vi "Base Probability calculation.vi"(8 "std [%]":dbl=0.02 format="%#_13g", 10 "Base Ex Info":T1, 11 "Relative Array":dbl[](array[numeric])) -> (3 "Time Probability":dbl[][](array[numeric]))   [LabVIEW 2018]
uses:
  <vilib>/gmath/statdist.llb/Normal PDF.vi
  <vilib>/gmath/NI_Gmath.lvlib
panel:
  out "Base R level":dbl[](array[numeric])
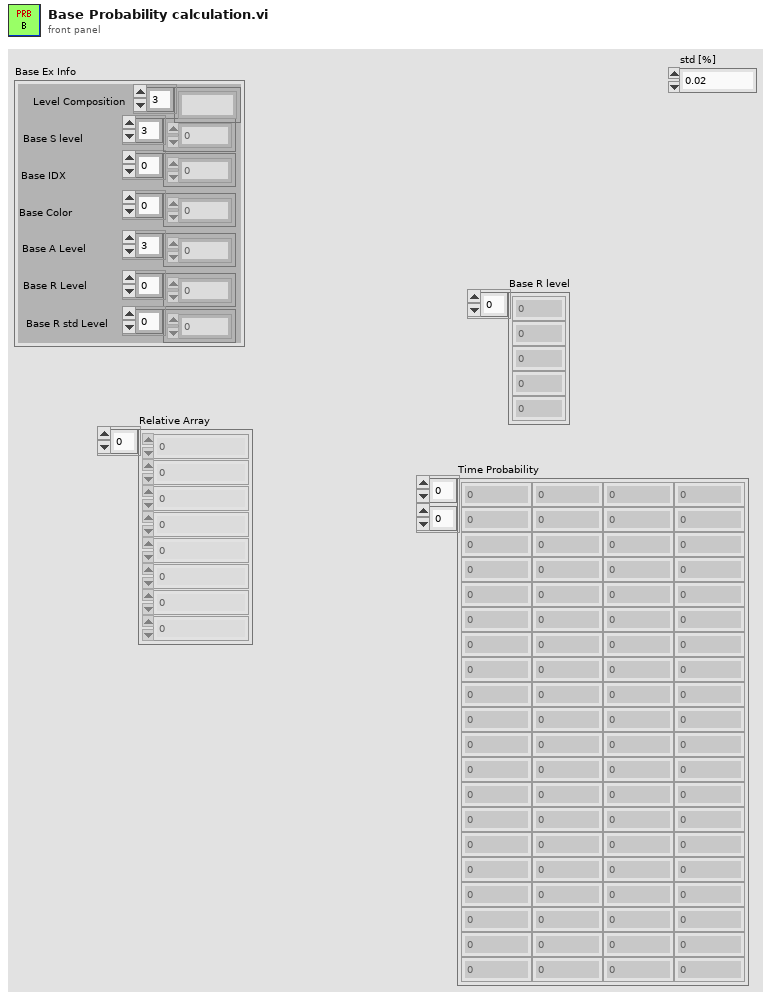
[diagram p1: front panel]
types:
  T1 = cluster{"Level Composition":string[], "Base S level":dbl[], "Base IDX":i32[], "Base Color":u32[], "Base A Level":dbl[], "Base R Level":dbl[], "Base R std Level":dbl[]}
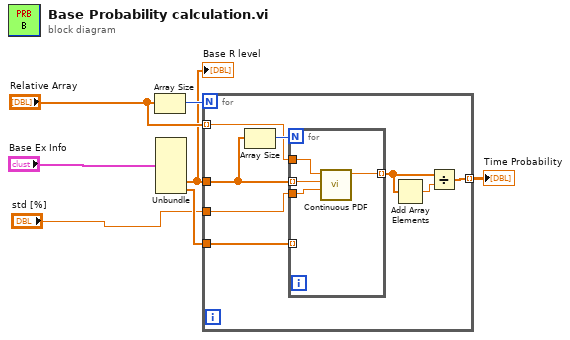
[diagram p0: block diagram]
diagram:
  n1 = Array Size(array="Relative Array") -> (size(s)=w7:i32)
  n2 = Unbundle("Base Ex Info") -> ("Base R Level"=w4:dbl[], "Base R std Level"=w2:dbl[])  [unwired: 5 out]
  "Base R level" <- w4
  n3 = for {
    N: w7 -> [_]
    tunnel: w4 -> [w14]
    tunnel: "Relative Array" -> [w13] mode=indexing
    tunnel: "std [%]" -> [w12]
    tunnel: [w9] -> w5 mode=indexing
    tunnel: w2 -> [w8]
    n4 = Array Size(array=w14) -> (size(s)=w15:i32)
    n5 = for {
      N: w15 -> [_]
      tunnel: w14 -> [w19] mode=indexing
      tunnel: w13 -> [w18]
      tunnel: w12 -> [w16]
      tunnel: [w17] -> w11 mode=indexing
      tunnel: w8 -> [_] mode=indexing
      n6 = call-poly <vilib>:"Continuous PDF.vi"("std"=w16, "mean"=w19, "x"=w18) -> ("pdf(x)"=w17:dbl)  [unwired: 7 in, 1 out]
    }
    n7 = Add Array Elements(numeric array=w11) -> (sum=w10:dbl)
    n8 = Divide(x=w11, y=w10) -> (x/y=w9:dbl[])
  }
  "Time Probability" <- w5
